vi "Save Image.vi"(8 "error in (no error)":errorcluster, 10 "Paths":path[](array[path]), 11 "ImageHandler:DT-ImageHandler in":refnum<class "DT-ImageHandler.lvclass">) -> (0 "error out":errorcluster, 3 "ImageHandler:DT-ImageHandler out":refnum<class "DT-ImageHandler.lvclass">)   [LabVIEW 2022 SP3, in "ImageHandler.lvlib" / "DT-ImageHandler.lvclass"]
uses:
  DT-ImageHandler.lvclass
  DT-ImageHandler.lvclass/DT-ImageHandler.ctl
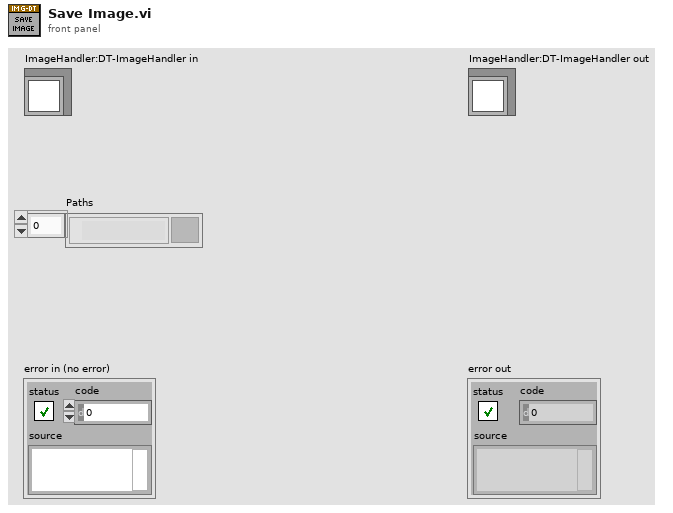
[diagram p1: front panel]
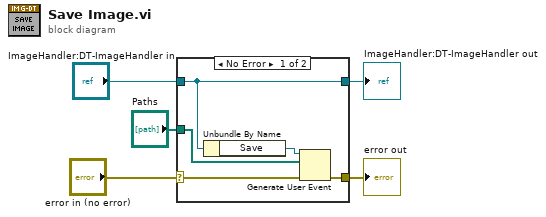
[diagram p0: block diagram]
diagram:
  n1 = case shown="No Error" "error in (no error)" {
    selector: "error in (no error)" -> [w7 w12]
    tunnel: [w6 w12] -> w4
    tunnel: [w10 w11] -> w2
    tunnel: "ImageHandler:DT-ImageHandler in" -> [w10 w11]
    tunnel: "Paths" -> [w8 _]
    frame No Error {
      n2 = Unbundle By Name(w10) -> ("Save"=w9:refnum<user-event>)
      n3 = Generate User Event(user event=w9, event data cluster=w8, error in=w7) -> (error out=w6:errorcluster)  [unwired: 1 in, 1 out]
    }
    frame Error {
    }
  }
  "error out" <- w4
  "ImageHandler:DT-ImageHandler out" <- w2
